vi "[ex ce] 4 Two-sides computation.vi"() -> ()   [LabVIEW 2021]
doc: "<B>Two-sides computation</B> (CE Client Example)\n\nThis example demonstrates how you can transfer data between expressions calculated on client and server sides. Advantage of this method is undependence of variable types. You can change name and type of variable at runtime without changing of a VI's Block Diagram.\n\nTo execute this example, you need run <B>\"[ex ce] CE Server Example.vi</B> on either local or remote computer. Also, you need <B>LabVIEW Advanced Analysis VIs</B> on server side.\n\n::: CalcExpress Toolkit :::\nCopyright (c) 2000-2026 Konstantin Shifershteyn. All rights reserved."
panel:
  in  "?":string="Name of variable is to used to transfer data from the client-side expression to server-side expression.\nAfter client's expression is computed, this variable is duplicated to a server and then is used to evaluate an expression on the server side.\nNote that it's possible to transfer variables of any datatype between client and server with the use of this technique."
  in  "var name":string="z" caption="Name of variable which is used for transferring data from client-side expression to server-side expression."
  out "Result":dbl[][](graph) caption="Result computed on server side"
  in  "remote expression":string="// Computes Magnitude of 2D FFT of 'x'\nnorm( fft2D(z) )\n"
  in  "To execute this example, you need run \"[ex ce] CE Server Example.vi\" on either local or remote computer. Also, you need the Advanced Analysis Libraries on server side.\n-------------------------------------------\nThis example demonstrates how you can transfer data between expressions calculated on client and server sides. Advantage of this method is independence of variable data types. You can change name and type of variable at runtime without changing of VI's Block Diagram.":string="To execute this example, you need run \"[ex ce] CE Server Example.vi\" on either local or remote computer. Also, you need the Advanced Analysis Libraries on server side.\n-------------------------------------------\nThis example demonstrates how you can transfer data between expressions calculated on client and server sides. Advantage of this method is independence of variable data types. You can change name and type of variable at runtime without changing of VI's Block Diagram."
  in  "use TCP for local":bool
  in  "local expression":string="x = nvecins (0, 64, 0.5); //1D: 0, 0.5 .. 31.5\nz = matrixn(0, 64, 64);  //2D: 64x64 of zero\nz += sin(x);             //each row == sin(x)\nz *= transp(z);          //row[i] * column[i]"
  out "Initial data":dbl[][](graph) caption="Data generated on client side"
  in  "port":u32=3363
  in  "machine name (empty = local)":string
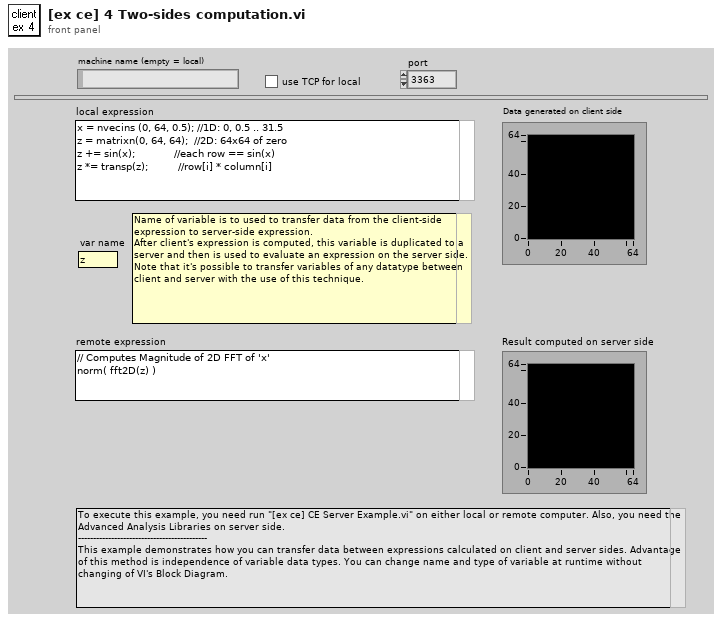
[diagram p1: front panel]
types:
  T1 = typedef "VarMan Variable Context Handle.ctl" = i32
  T2 = typedef "CE Session.ctl" = cluster{"VI refnum":refnum<vi>, "VC Handle":T1}
  T3 = typedef "CalcExpress Data Type.ctl" = enum32{"String", "DBL Number", "identifier", "1D Array of DBL", "2D Array of DBL", "CDB Number", "1D Array of CDB", "2D Array of CDB", "1D Array of String", "2D Array of String", "Unknown data type"}
  T4 = cluster{"type":T3, "dbl":dbl, "cdb":cdb, "str":string, "1d dbl":dbl[], "1d cdb":cdb[], "1d str":string[], "2d dbl":dbl[][], "2d cdb":cdb[][], "2d str":string[][]}
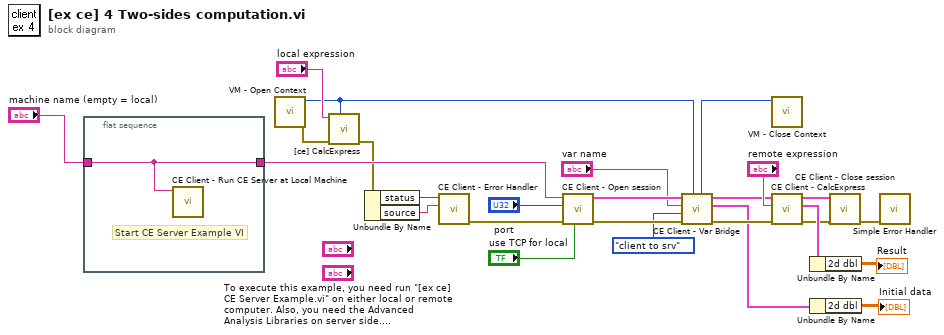
[diagram p0: block diagram]
diagram:
  n1 = flat-sequence {
    tunnel: [w27] -> w7
    tunnel: "machine name (empty = local)" -> [w27]
    frame #0 {
      # "Start CE Server Example VI"
      n2 = call "CE Client - Run CE Server at Local Machine.vi"("machine name"=w27) -> ()  [unwired: 9 in, 2 out]
    }
  }
  n3 = call "VM - Open Context.vi"() -> ("error out"=w5:errorcluster, "VC Handle out"=w12:T1)  [unwired: 9 in, 1 out]
  n4 = call "[ce] CalcExpress.vi"("VC Handle"=w12, "error in"=w5, "expression"="local expression") -> ("error out"=w4:errorcluster)  [unwired: 3 in, 3 out]
  n5 = Unbundle By Name(w4) -> ("status"=w3:bool, "source"=w2:string)
  n6 = call "CE Client - Error Handler.vi"("error message"=w2, "CE error status"=w3) -> ("error out"=w8:errorcluster)  [unwired: 7 in]
  n7 = call "CE Client - Open session.vi"("use TCP for local (F)"="use TCP for local", "error in"=w8, "port number (3363)"="port", "machine name (empty - local)"=w7) -> ("error out"=w11:errorcluster, "CE session out"=w10:T2)  [unwired: 4 in]
  n8 = call "CE Client - Var Bridge.vi"("local VC Handle"=w12, "error in"=w11, "direction"=enum16{"client to srv", "srv to client"}."client to srv", "var name"="var name", "CE session"=w10) -> ("error out"=w17:errorcluster, "values out"=w15:T4, "dup CE session"=w16:T2, "dup local VC Handle"=w13:T1)  [unwired: 3 in]
  n9 = call "VM - Close Context.vi"("VC Handle"=w13) -> ()  [unwired: 9 in, 2 out]
  n10 = call "CE Client - CalcExpress.vi"("error in"=w17, "expression"="remote expression", "CE session"=w16) -> ("error out"=w21:errorcluster, "values out"=w23:T4, "dup CE session"=w22:T2)  [unwired: 4 in]
  n11 = Unbundle By Name(w23) -> ("2d dbl"=→"Result":dbl[][])
  n12 = Unbundle By Name(w15) -> ("2d dbl"=→"Initial data":dbl[][])
  n13 = call "CE Client - Close session.vi"("error in"=w21, "CE session"=w22) -> ("error out"=w24:errorcluster)  [unwired: 6 in, 1 out]
  n14 = call <vilib>:"Simple Error Handler.vi"("error in (no error)"=w24) -> ()  [unwired: 4 in, 5 out]
